vi "Strip Trailing Zeros for Float String.vi"(11 "Float String":string) -> (3 "Float String with Same Value":string)   [LabVIEW 2017, in "API String Arguments Support.lvlib"]
uses:
  API String Arguments Support.lvlib
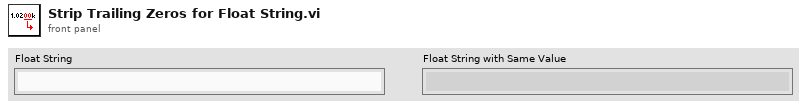
[diagram p1: front panel]
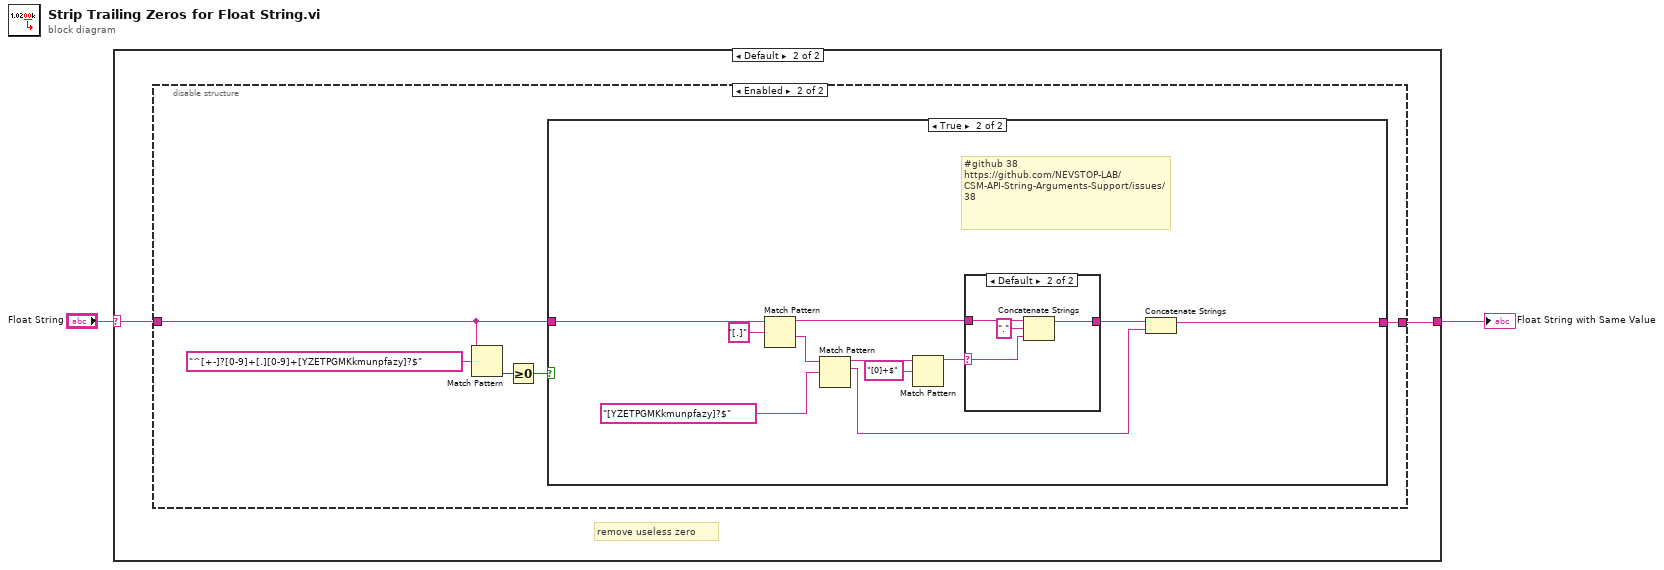
[diagram p0: block diagram]
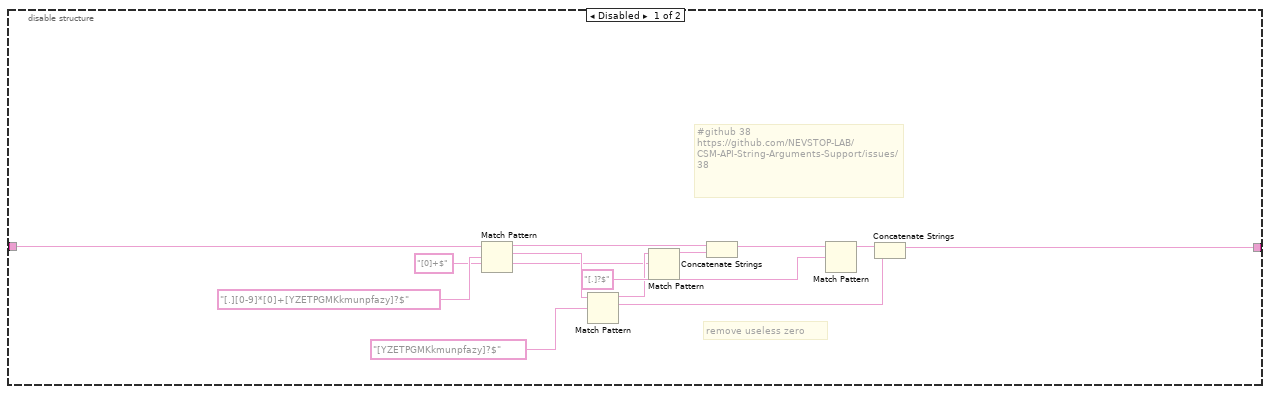
[diagram p3: hidden frame]
diagram:
  n1 = case shown="Default" "Float String" {
    selector: "Float String" -> [w3 w4]
    tunnel: [w3 w5] -> w2
    frame "", "-Inf", "e", "Inf", "NaN", "pi" {
    }
    frame Default {
      # "remove useless zero"
      n2 = disable-structure shown="Enabled" {
        disable-tunnel: [w18 w23] -> w5
        disable-tunnel: w4 -> [w14 w21]
        frame Disabled {
          # "#github 38\nhttps://github.com/NEVSTOP-LAB/CSM-API-String-Arguments-Support/issues/38"
          # "remove useless zero"
          n3 = Match Pattern(string=w14, regular expression="[.][0-9]*[0]+[YZETPGMKkmunpfazy]?$") -> (before substring=w15:string, match substring=w17:string)  [unwired: 1 in, 2 out]
          n4 = Match Pattern(string=w17, regular expression="[YZETPGMKkmunpfazy]?$") -> (before substring=w9:string, match substring=w10:string)  [unwired: 1 in, 2 out]
          n5 = Match Pattern(string=w9, regular expression="[0]+$") -> (before substring=w8:string)  [unwired: 1 in, 3 out]
          n6 = Concatenate Strings(w15, w8) -> (w12:string)
          n7 = Match Pattern(string=w12, regular expression="[.]?$") -> (before substring=w13:string)  [unwired: 1 in, 3 out]
          n8 = Concatenate Strings(w13, w10) -> (w18:string)
        }
        frame Enabled {
          n9 = Match Pattern(string=w21, regular expression="^[+-]?[0-9]+[.][0-9]+[YZETPGMKkmunpfazy]?$") -> (offset past match=w20:i32)  [unwired: 1 in, 3 out]
          n10 = Greater Or Equal To 0?(x=w20) -> (x >= 0?=w19:bool)
          n11 = case shown="True" w19 {
            tunnel: [w24 w35] -> w23
            tunnel: w21 -> [w24 w30]
            frame False {
            }
            frame True {
              # "#github 38\nhttps://github.com/NEVSTOP-LAB/CSM-API-String-Arguments-Support/issues/38"
              n12 = Match Pattern(string=w30, regular expression="[.]") -> (before substring=w33:string, after substring=w31:string)  [unwired: 1 in, 2 out]
              n13 = Match Pattern(string=w31, regular expression="[YZETPGMKkmunpfazy]?$") -> (before substring=w26:string, match substring=w25:string)  [unwired: 1 in, 2 out]
              n14 = Match Pattern(string=w26, regular expression="[0]+$") -> (before substring=w27:string)  [unwired: 1 in, 3 out]
              n15 = case shown="Default" w27 {
                selector: w27 -> [_ w37]
                tunnel: [w36 w40] -> w29
                tunnel: w33 -> [w36 w38]
                frame "" {
                }
                frame Default {
                  n16 = Concatenate Strings(w38, "." ("regular expression"), w37) -> (w40:string)
                }
              }
              n17 = Concatenate Strings(w29, w25) -> (w35:string)
            }
          }
        }
      }
    }
  }
  "Float String with Same Value" <- w2
